vi "Base sp cluster selection for database.vi"(8 "error in":errorcluster, 11 "Base":string) -> (0 "error out":errorcluster, 1 "Item":T1, 2 "element":string="000.csv", 3 "Base Species IDX":i32)   [LabVIEW 2018]
panel:
  out "R STD Level":dbl
  out "R Base Level":dbl
  out "Base Color":u32
  out "ex":string
  out "index":i32
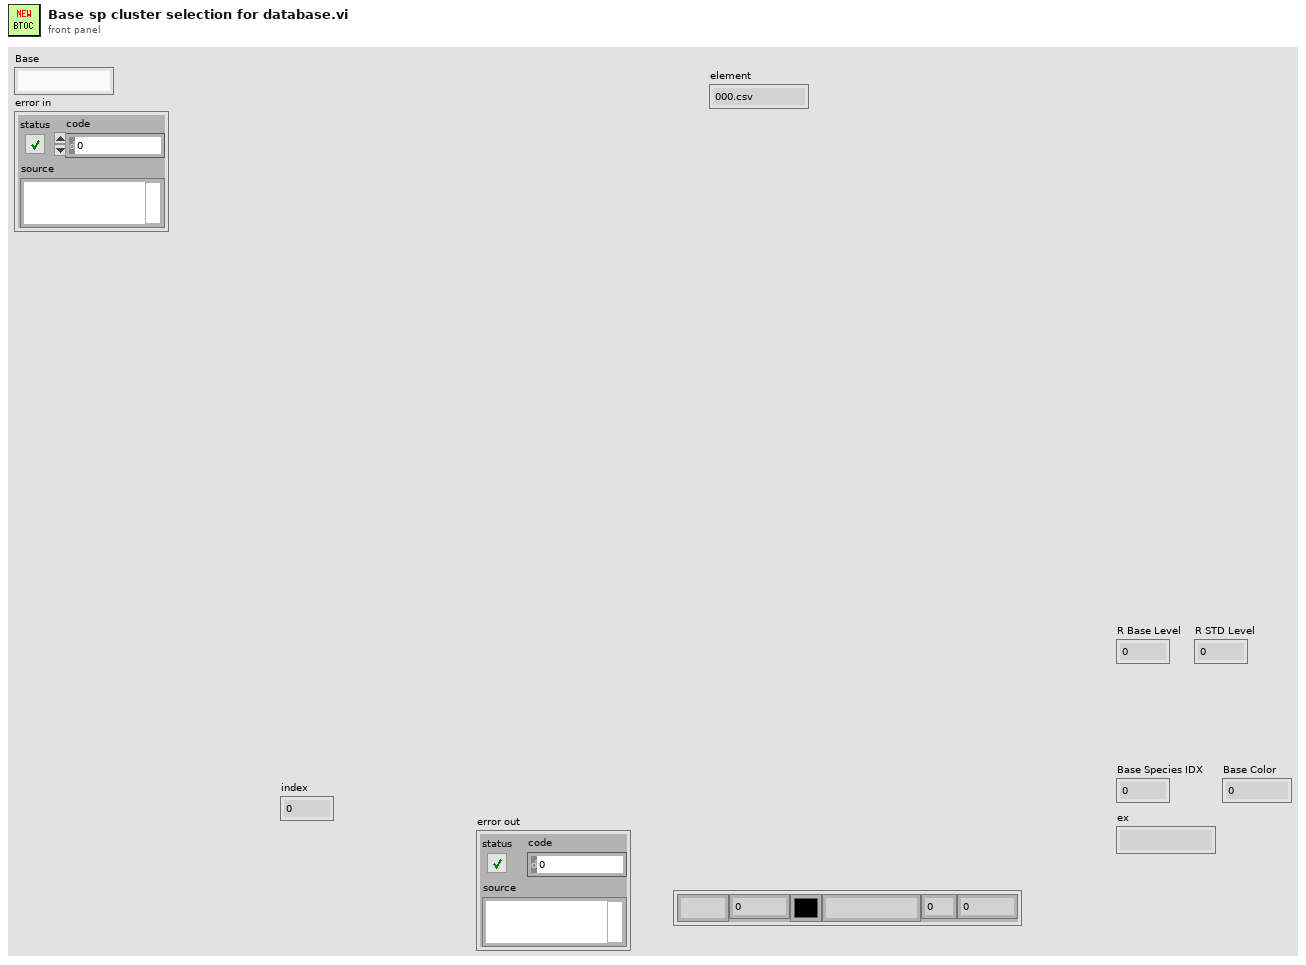
[diagram p1: front panel]
types:
  T1 = cluster{"Name":string, "Value":dbl, "Color":u32, "Name 2":string, "Value 2":dbl, "Value 3":dbl}
  T2 = cluster{"String":string, dbl, i32, "String":string, i32, dbl}
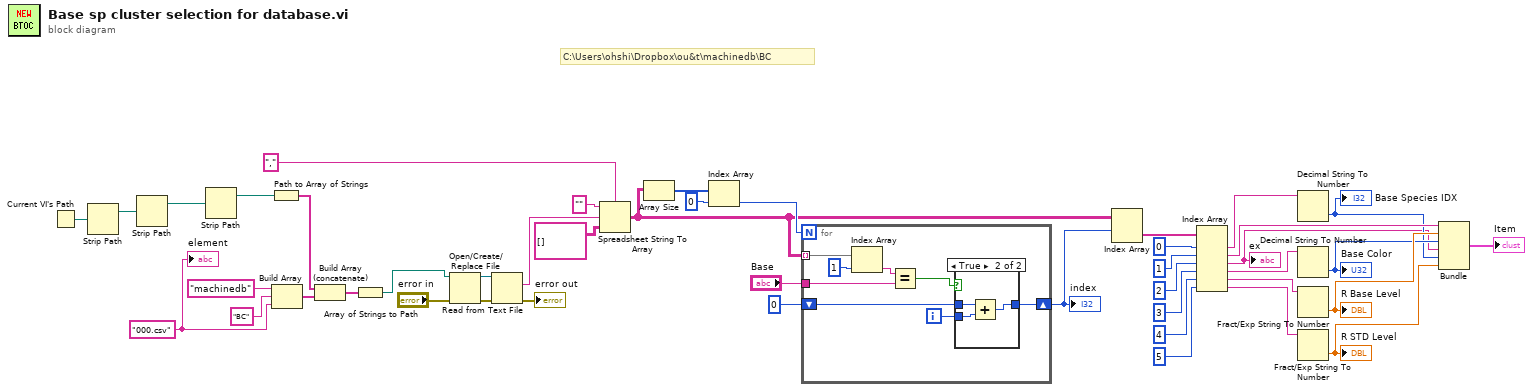
[diagram p0: block diagram]
diagram:
  w38 = "000.csv" ("element")
  # "C:\\Users\\ohshi\\Dropbox\\ou&t\\machinedb\\BC"
  n1 = Current VI's Path() -> (path=w44:path)
  n2 = Strip Path(path=w44) -> (stripped path=w43:path)  [unwired: 1 out]
  n3 = Strip Path(path=w43) -> (stripped path=w42:path)  [unwired: 1 out]
  n4 = Strip Path(path=w42) -> (stripped path=w41:path)  [unwired: 1 out]
  n5 = Path to Array of Strings(0:w41) -> (2:w37:string[])  [unwired: 1 out]
  n6 = Build Array("machinedb", "BC", w38) -> (w36:string[])
  n7 = Build Array (concatenate)(w37, w36) -> (w35:string[])
  n8 = Array of Strings to Path(0:w35) -> (2:w34:path)  [unwired: 1 in]
  n9 = Open/Create/Replace File(file path (use dialog)=w34, error in="error in") -> (refnum out=w31:refnum<file>, error out=w32:errorcluster)  [unwired: 4 in, 1 out]
  n10 = Read from Text File(file (use dialog)=w31, error in=w32) -> (text=w30:string, error out=→"error out":errorcluster)  [unwired: 2 in, 2 out]
  n11 = Spreadsheet String To Array(delimiter (Tab)=",", format string="", spreadsheet string=w30, array type (2D Dbl)=string[][] []) -> (array=w19:string[][])
  n12 = Array Size(array=w19) -> (size(s)=w25:i32[])
  n13 = Index Array(array=w25, index=0) -> (element=w23:i32)
  n14 = for {
    N: w23 -> [_]
    tunnel: w19 -> [w52] mode=indexing
    tunnel: "Base" -> [w49]
    shift-right: [w46] -> w20
    shift-left: 0 ("index") -> [w47]
    i -> [w45]
    n15 = Index Array(array=w52, index=1) -> (element=w50:string)
    n16 = Equal?(x=w50, y=w49) -> (x = y?=w48:bool)
    n17 = case shown="True" w48 {
      tunnel: [w53 w55] -> w46
      tunnel: w47 -> [w53 w54]
      tunnel: w45 -> [_ w56]
      frame False {
      }
      frame True {
        n18 = Add(x=w54, y=w56) -> (x+y=w55:i32)
      }
    }
  }
  "index" <- w20
  n19 = Index Array(array=w19, index (row)=w20) -> (element=w18:string[])  [unwired: 1 in]
  n20 = Index Array(array=w18, index #1=0 ("index"), index #2=1 ("index"), index #3=2 ("index"), index #4=3 ("index"), index #5=4 ("index"), index #6=5 ("index")) -> (element #1=w16:string, element #2=w14:string, element #3=w1:string, element #4=w8:string, element #5=w10:string, element #6=w5:string)
  "ex" <- w1
  n21 = Decimal String To Number(string=w16) -> (number=w4:i32)  [unwired: 2 in, 1 out]
  "Base Species IDX" <- w4
  n22 = Decimal String To Number(string=w8) -> (number=w7:i32)  [unwired: 2 in, 1 out]
  "Base Color" <- w7
  n23 = Fract/Exp String To Number(string=w10) -> (number=w9:dbl)  [unwired: 3 in, 1 out]
  "R Base Level" <- w9
  n24 = Fract/Exp String To Number(string=w5) -> (number=w2:dbl)  [unwired: 3 in, 1 out]
  "R STD Level" <- w2
  n25 = Bundle("String"=w14, w9, w7, "String"=w1, w4, w2) -> (→"Item":T2)  [unwired: 1 in]
  "element" <- w38
